vi "Update External Clock.vi"(8 "error in (no error)":errorcluster, 11 "CAN_Reader_NIXNET":refnum<class "CAN_Reader_CANsub_Plugin.lvclass">) -> (0 "error out":errorcluster, 3 "CAN_Reader_NIXNET":refnum<class "CAN_Reader_CANsub_Plugin.lvclass">)   [LabVIEW 2021, in "CAN_Reader_CANsub_Plugin.lvclass"]
uses:
  CAN_Reader_CANsub_Plugin.lvclass
  CAN_Reader_CANsub_Plugin.lvclass/CAN_Reader_CANsub_Plugin.ctl
  <vilib>/CIF Foundation/CIF XNET CAN RW/XNET CAN RW.lvclass
  <vilib>/CIF Foundation/CIF Core/CIFCore/Class/CIFCorePlugin.lvclass
  <vilib>/CIF Foundation/CIF Utilities/Time/Typedef/Timestamp Pair.ctl
  <vilib>/CIF Foundation/CIF Utilities/Time/Time_CIF_U.lvlib
  C:/Program Files/National Instruments/LabVIEW 2021/vi.lib/CIF Foundation/CIF Core/CIFCore/Class/CIFCorePlugin.lvclass
  D:/dev/Plugins/CAN_Reader_CANsub/Class/CAN_Reader_CANsub_Plugin.lvclass
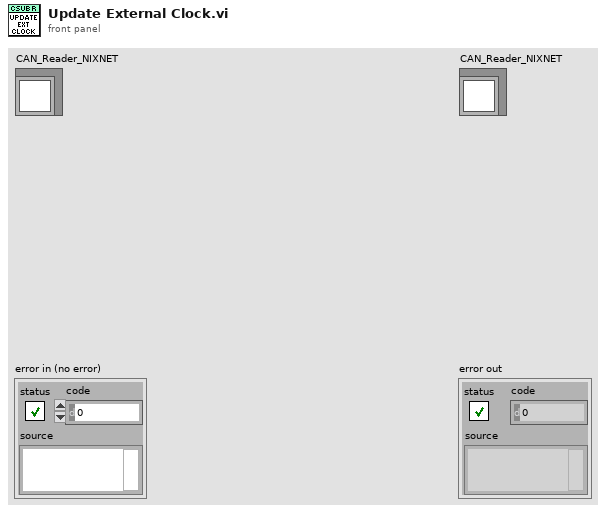
[diagram p1: front panel]
types:
  T1 = typedef "Time_CIF_U.lvlib/Timestamp Pair.ctl" = cluster{"System Time":i64, "External Time":i64}
  T2 = typedef "XNET CAN RW.lvclass/Time Pair.ctl" = cluster{"System Time":i64, "CAN Time":i64}
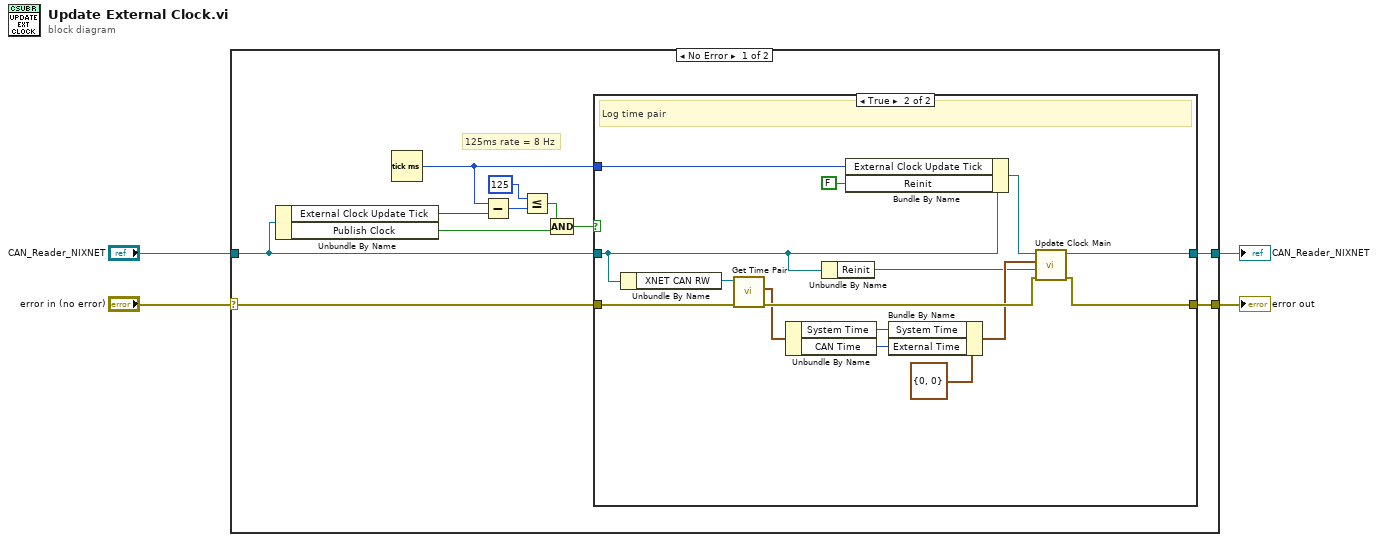
[diagram p0: block diagram]
diagram:
  n1 = case shown="No Error" "error in (no error)" {
    selector: "error in (no error)" -> [w7 w34]
    tunnel: [w6 w34] -> w3
    tunnel: [w8 w33] -> w1
    tunnel: "CAN_Reader_NIXNET" -> [w15 w33]
    frame No Error {
      # "125ms rate = 8 Hz"
      n2 = Unbundle By Name(w15) -> ("External Clock Update Tick"=w14:u32, "Publish Clock"=w13:bool)
      n3 = Tick Count (ms)() -> (millisecond timer value=w5:u32)
      n4 = Subtract(x=w5, y=w14) -> (x-y=w11:u32)
      n5 = Less Or Equal?(x=u32 125 ("x-y"), y=w11) -> (x <= y?=w9:bool)
      n6 = Compound Arithmetic op=AND(w9, w13) -> (w12:bool)
      n7 = case shown="True" w12 {
        tunnel: w15 -> [w16 w19]
        tunnel: [w16 w31] -> w8
        tunnel: w7 -> [w17 w29]
        tunnel: [w17 w28] -> w6
        tunnel: w5 -> [_ w26]
        frame False {
          # "Don't update (not enable or recently updated)"
        }
        frame True {
          # "Log time pair"
          n8 = Unbundle By Name(w19) -> ("XNET CAN RW"=w32:refnum<class "XNET CAN RW.lvclass">)
          n9 = call <vilib>:"Get Time Pair.vi"("error in (no error)"=w29, "XNET CAN RW in"=w32) -> ("error out"=w30:errorcluster, "Time Pair"=w22:T2)  [unwired: 7 in, 1 out]
          n10 = Unbundle By Name(w22) -> ("System Time"=w21:i64, "CAN Time"=w20:i64)
          n11 = Unbundle By Name(w19) -> ("Reinit"=w18:bool)
          n12 = Bundle By Name(cluster=w19, "External Clock Update Tick"=w26, "Reinit"=FALSE ("External Clock Controls.Reinit")) -> (w27:refnum<class "CAN_Reader_CANsub_Plugin.lvclass">)
          n13 = Bundle By Name(cluster=T1 {"System Time"=0, "External Time"=0} ("Timestamp Pair"), "System Time"=w21, "External Time"=w20) -> (w23:T1)
          n14 = call <vilib>:"Update Clock Main.vi"("error in (no error)"=w30, "Reinit"=w18, "Timestamp Pair"=w23, "CIFCorePlugin in"=w27) -> ("error out"=w28:errorcluster, "CIFCorePlugin out"=w31:refnum<class "CAN_Reader_CANsub_Plugin.lvclass">)  [unwired: 6 in]
        }
      }
    }
    frame Error {
    }
  }
  "error out" <- w3
  "CAN_Reader_NIXNET" <- w1
